vi "fifo_experiment.lv2020.vi"(8 "fifo name":string="EXP-Fifo", 9 "vi name":string="fifo_scratch.vi", 10 "target name":string="FPGA Target", 11 "project path":string) -> (0 "error out":errorcluster, 2 "fifo item name":string, 3 "succeeded":bool)   [LabVIEW 2020]
doc: "One-FIFO scripting experiment (2026-10-16). Opens the project at project path, finds the project item named target name (the FPGA target) and the VI item named vi name under it, creates a target-scoped U64 FIFO named fifo name with the given depth through NI's unsupported FPGA scripting API (vi.lib\\rvi\\ClientSDK\\Core\\Script\\Fifo), commits it to the project, drops the FIFO Method Node for it onto the VI's block diagram (nirvififoDropXNodeFromProject.vi), saves the VI and the project and closes the project. succeeded = the node drop reported success."
panel:
  out "vi index":i32
  out "target index":i32
  out "item count":i32
  out "name read errors":errorcluster[](array[cluster])
  in  "depth":u32=1024
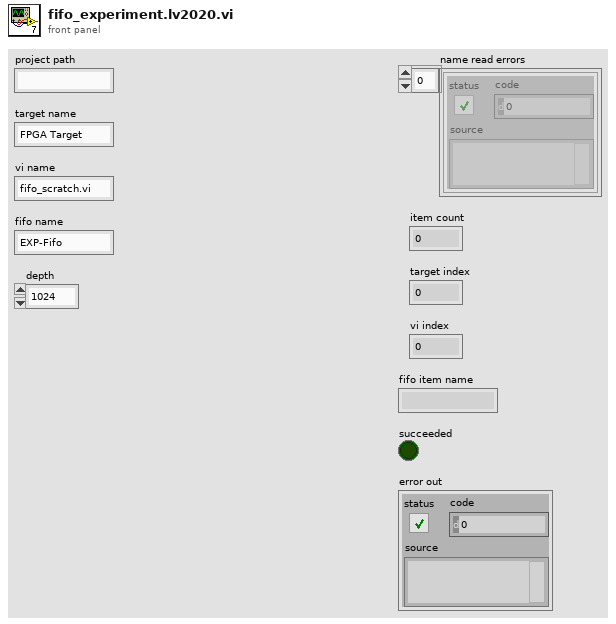
[diagram p1: front panel]
types:
  T1 = enum16{"Target-Scoped", "Host to Target - DMA", "Target to Host - DMA", "Peer to Peer Reader", "Peer to Peer Writer"}
  T2 = typedef "nirviPiFifo_State.ctl" = cluster{"Item":refnum<vi>, "Fifo":T3, "Dirty":bool, "XNode":refnum<vi>}
  T3 = typedef "niFpgaContainerState.ctl" = cluster{"displayName":string, "hardwareName":string, "dataType":T4, "elementTypeDescriptor":variant, "terminalTypeDescriptor":variant, "requestedNumberOfElements":u32, "memoryType":T5, "arbitrationForInterfaceA":T6, "numberOfElementsPerRead":u32, "arbitrationForInterfaceB":T6, "numberOfElementsPerWrite":u32, "VI_Defined":bool, "type":T7, "initializationParameters":T8, "disableOnOverflow/Underflow":bool, "interfaceConfiguration":T9, "controlLogic":T10, "actualNumberOfElements":u32, "dramSelection":string, "dramMaxOustandingRequests":i32, "dramIncludeByteEnables":bool, "dramGrantTime":u32, "fullEmulation":bool, "memoryInMultipleClockDomains":bool, "memoryLatency":T11}
  T4 = typedef "niFpgaDataTypeControl.ctl" = enum32{"Boolean", "I8", "I16", "I32", "I64", "U8", "U16", "U32", "U64", "FXP", "CustomControl", "SGL"}
  T5 = typedef "niFpgaContainerImplementationControl.ctl" = enum16{"Flip-Flops", "Look-Up Table", "Block Memory", "DRAM", "UltraRAM"}
  T6 = typedef "niFpgaContainerArbitrationOptionsControl.ctl" = enum16{"Always Arbitrate", "Arbitrate if Multiple Requestors Only", "Never Arbitrate"}
  T7 = typedef "niFpgaTransferTypeControl.ctl" = enum16{"Target-Scoped", "Host to Target - DMA", "Target to Host - DMA", "Peer to Peer Reader", "Peer to Peer Writer", "Bidirectional", "Memory Buffer Reader", "Memory Buffer Writer"}
  T8 = typedef "niFpgaContainerInitializationParameters.ctl" = cluster{"initialized":bool, "VI_Path":path, "initialData":variant}
  T9 = typedef "niFpgaMemoryInterfaceConfiguration.ctl" = enum16{"Read A-Write B", "Read A-Read B"}
  T10 = typedef "niFpgaFifoControlLogicControl.ctl" = enum16{"Slice Fabric", "Target Optimal", "Built-in"}
  T11 = typedef "niFpgaContainerMemoryLatencyControl.ctl" = u16
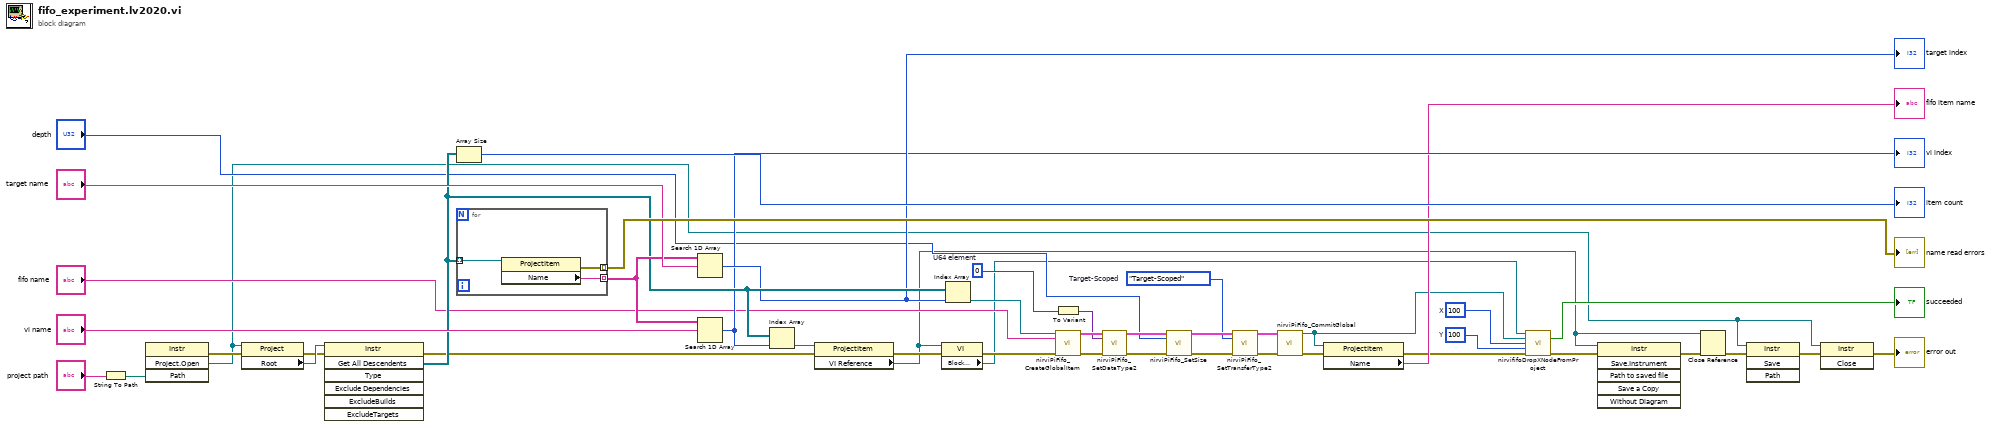
[diagram p0: block diagram]
diagram:
  w10 = 100  # Y
  w11 = 100  # X
  w19 = T1."Target-Scoped"  # Target-Scoped
  w27 = u64 0  # U64 element
  n1 = String To Path(string="project path") -> (path=w45:path)
  n2 = invoke class="Instr" method="Project.Open"("Path"=w45) -> (error out=w44:errorcluster, "Project:Open"=w3:refnum<vi>)  [unwired: 3 in, 2 out]
  n3 = property class="Project"(reference=w3, error in=w44) -> (error out=w42:errorcluster, "Root"=w43:refnum<vi>)  [unwired: 1 out]
  n4 = invoke class="Instr" method="Get All Descendents"(reference=w43, error in=w42) -> (error out=w32:errorcluster, "All Descendents"=w36:refnum<vi>[])  [unwired: 5 in, 5 out]
  n5 = Array Size(array=w36) -> (size(s)=→"item count":i32)
  n6 = for {
    tunnel: w36 -> [w49] mode=indexing
    tunnel: [w48] -> w38 mode=indexing
    tunnel: [w47] -> w41 mode=indexing
    n7 = property class="ProjectItem"(reference=w49) -> (error out=w47:errorcluster, "Name"=w48:string)  [unwired: 1 in, 1 out]
  }
  "name read errors" <- w41
  n8 = Search 1D Array(1D array=w38, element="target name") -> (index of element=w35:i32)  [unwired: 1 in]
  "target index" <- w35
  n9 = Search 1D Array(1D array=w38, element="vi name") -> (index of element=w34:i32)  [unwired: 1 in]
  "vi index" <- w34
  n10 = Index Array(array=w36, index=w34) -> (element=w33:refnum<vi>)
  n11 = property class="ProjectItem"(reference=w33, error in=w32) -> (error out=w31:errorcluster, "VI Reference"=w6:refnum<vi>)  [unwired: 1 out]
  n12 = property class="VI"(reference=w6, error in=w31) -> (error out=w28:errorcluster, "Block Diagram"=w13:refnum<vi>)  [unwired: 1 out]
  n13 = Index Array(array=w36, index=w35) -> (element=w30:refnum<vi>)
  n14 = call <vilib>:"nirviPiFifo_CreateGlobalItem.vi"("parent item"=w30, "name"="fifo name", "error in (no error)"=w28) -> ("reference"=w26:T2, "error out"=w24:errorcluster)  [unwired: 11 in]
  n15 = To Variant(anything=w27) -> (Variant=w25:variant)
  n16 = call <vilib>:"nirviPiFifo_SetDataType2.vi"("Reference"=w26, "Data Type"=w25, "error in (no error)"=w24) -> ("Reference"=w23:T2, "error out"=w21:errorcluster)  [unwired: 11 in]
  n17 = call <vilib>:"nirviPiFifo_SetSize.vi"("Reference"=w23, "Size"="depth", "error in (no error)"=w21) -> ("Reference"=w20:T2, "error out"=w18:errorcluster)  [unwired: 11 in]
  n18 = call <vilib>:"nirviPiFifo_SetTransferType2.vi"("Reference"=w20, "Transfer Type"=w19, "error in (no error)"=w18) -> ("Reference"=w17:T2, "error out"=w16:errorcluster)  [unwired: 11 in]
  n19 = call <vilib>:"nirviPiFifo_CommitGlobal.vi"("Reference"=w17, "error in (no error)"=w16) -> ("ProjectItem"=w12:refnum<vi>, "error out"=w15:errorcluster)  [unwired: 12 in]
  n20 = property class="ProjectItem"(reference=w12, error in=w15) -> (error out=w9:errorcluster, "Name"=→"fifo item name":string)  [unwired: 1 out]
  n21 = call <vilib>:"nirvififoDropXNodeFromProject.vi"("Scratch Diagram"=w13, "Fifo ProjectItem"=w12, "X"=w11, "Y"=w10, "error in (no error)"=w9) -> ("Succeeded"=→"succeeded":bool, "error out"=w7:errorcluster)  [unwired: 8 in, 1 out]
  n22 = invoke class="Instr" method="Save.Instrument"(reference=w6, error in=w7) -> (error out=w5:errorcluster)  [unwired: 4 in, 5 out]
  n23 = Close Reference(reference=w6, error in (no error)=w5) -> (error out=w4:errorcluster)
  n24 = invoke class="Instr" method="Save"(reference=w3, error in=w4) -> (error out=w2:errorcluster)  [unwired: 2 in, 3 out]
  n25 = invoke class="Instr" method="Close"(reference=w3, error in=w2) -> (error out=→"error out":errorcluster)  [unwired: 1 in, 2 out]
